vi "uRedPC.vi"() -> ()   [LabVIEW 2019]
uses:
  <vilib>/addons/_office/excel.llb/Excel Get Data ([dbl]).vi
  <vilib>/Utility/NIReport.llb/NI_report.lvclass
  <vilib>/Utility/NIReport.llb/Excel/NI_Excel.lvclass
  <vilib>/addons/_office/NI_ReportGenerationToolkit.lvlib
panel:
  out "Time":u32
  in  "Tab Control":enum32{"SoC", "Voltge-Current"}(tab)
  out "SoC Vehiculo":dbl[](graph)
  out "Battery Voltage":dbl[](graph)
  out "Battery Current":dbl[](graph)
  in  "%C":dbl=0.5 min=0.0 max=0.5 step=0.01
  out "Pot_cons":dbl
  out "V_bat":dbl
  out "I_bat":dbl
  in  "SoC0_Vehiculo":dbl=0.4 min=0.0 max=1.0 step=0.001
  in  "Cargar":bool
  in  "Boolean":bool
  out "Potencia consumida":dbl
  in  "Falla PV":bool
  in  "SoC_ini":dbl=0.5 min=0.0 max=1.0 step=0.1
  in  "Numero Paneles":u8=4 step=1
  in  "Voltaje Red":dbl=120.0 min=0.0 max=240.0 step=120.0
  out "Perdida Batería":dbl
  out "Perdida PV":dbl
  in  "Numero Baterías":u8=4 min=1 step=1
  out "Ring":u16(ring)
  out "Sheet 1 Data 2":dbl[][](array[numeric]) format="%.2f"
  out "Irradiancia":dbl(graph)
  out "Sheet 1 Data":dbl[][](array[numeric]) format="%.2f"
  out "SoC":dbl[](graph)
  out "Potencias":T1(graph)
  in  "stop":bool
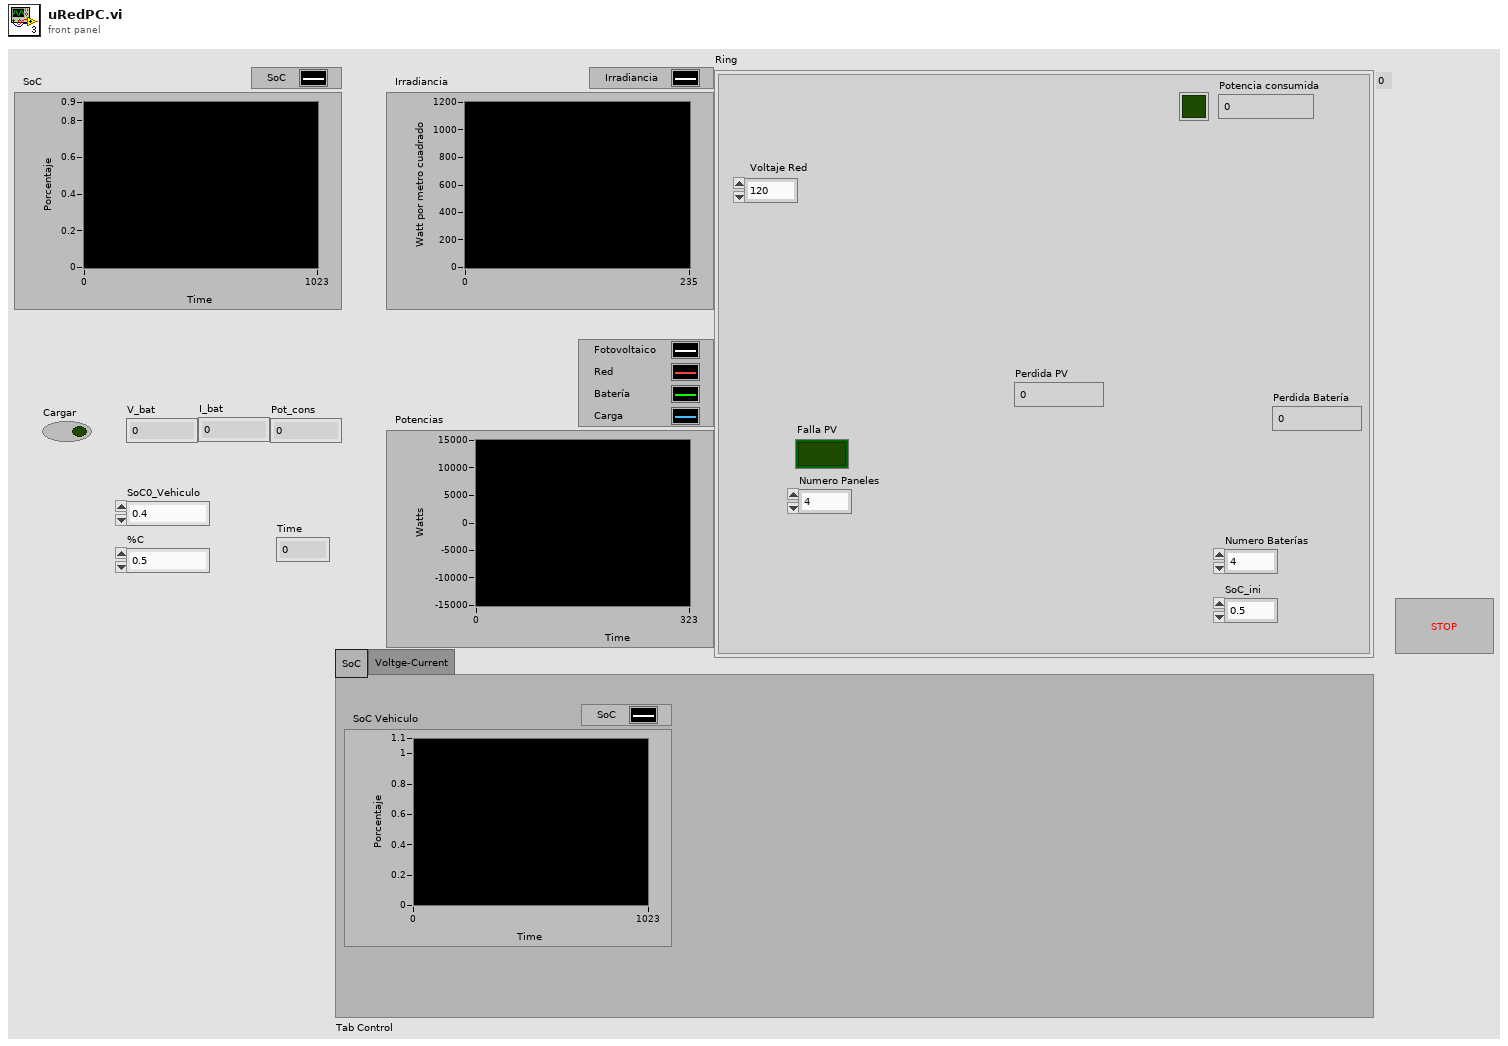
[diagram p1: front panel]
types:
  T1 = cluster{"Double":dbl, "Double":dbl, "Double":dbl, dbl}
  T2 = enum16{"Standard Report", "HTML", "Word", "Excel"}
  T3 = enum16{"open", "open or create", "create or replace", "create", "open (read-only)"}
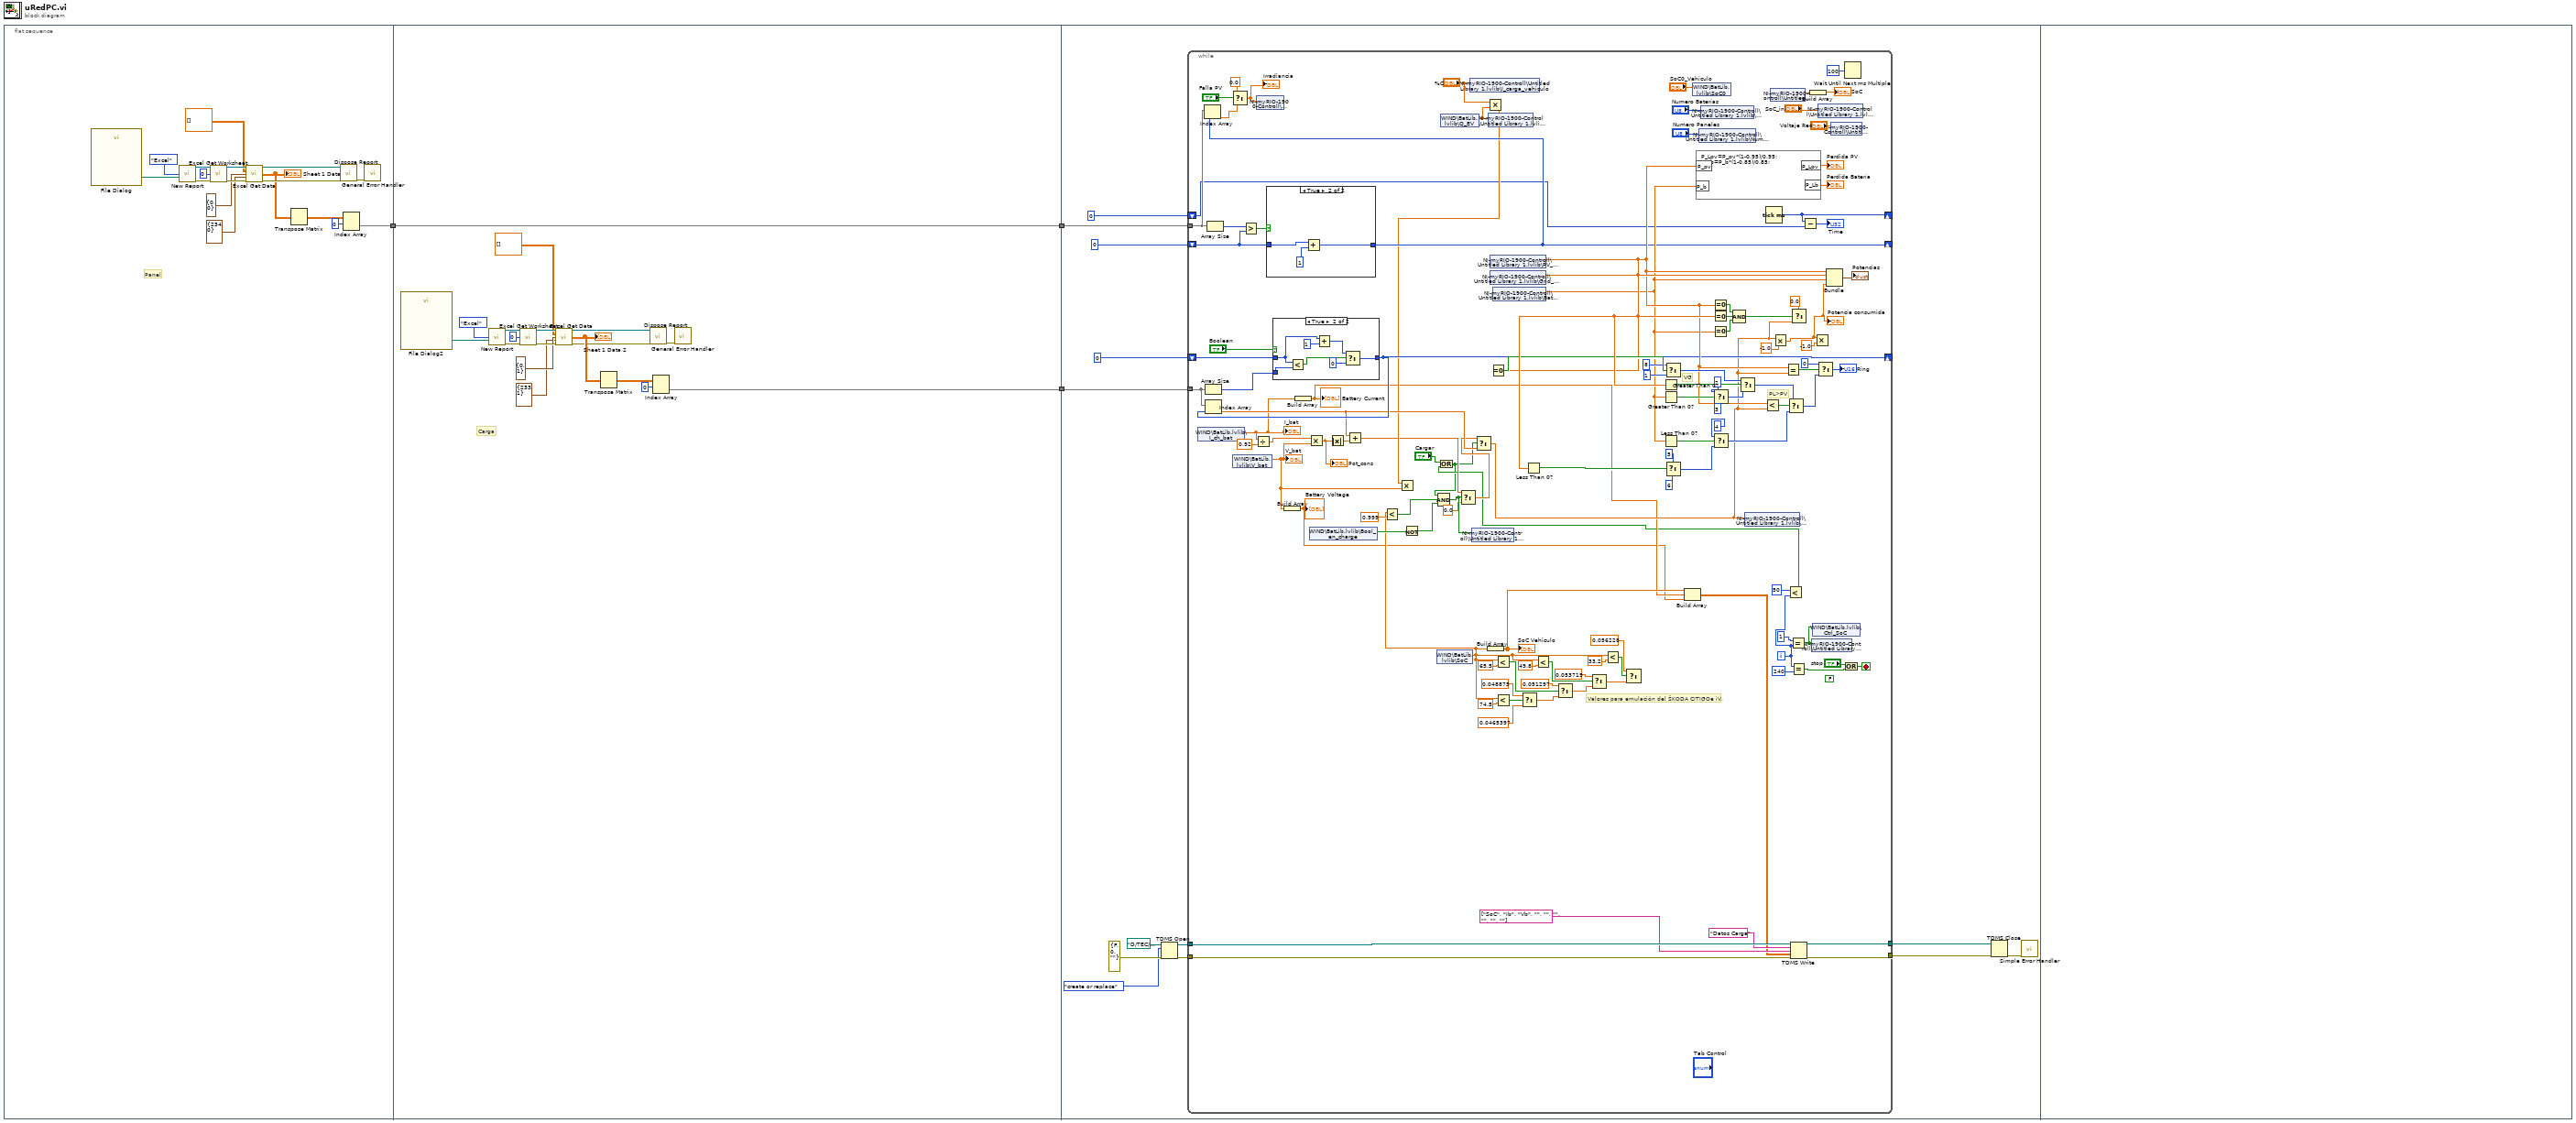
[diagram p0: block diagram]
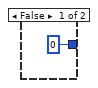
[diagram p3: hidden frame]
diagram:
  n1 = flat-sequence {
    tunnel: [w4] -> w3
    tunnel: [w38] -> w2
    tunnel: [w37] -> w1
    tunnel: w3 -> [w38]
    tunnel: w2 -> [w51]
    tunnel: w1 -> [w49]
    frame #0 {
      # "Panel"
      n2 = call "File Dialog"() -> ("selected path"=w11:path)  [unwired: 7 in, 8 out]
      n3 = call <vilib>:"New Report.vi"("report type"=T2."Excel", "template (empty)"=w11) -> ("report out"=w20:refnum<class "NI_report.lvclass">, "error out"=w16:errorcluster)  [unwired: 4 in, 8 out]
      n4 = call <vilib>:"Excel Get Worksheet.vi"("report in"=w20, "worksheet index (0)"=0, "error in (no error)"=w16) -> ("report out"=w19:refnum<class "NI_report.lvclass">, "error out"=w15:errorcluster)  [unwired: 11 out]
      n5 = call-poly <vilib>:"Excel Get Data.vi"("report in"=w19, "data type"=dbl[][] [], "start (-1, -1)"=cluster{"row":i32, "column":i32} {"row"=0, "column"=0}, "end (-1, -1)"=cluster{"row":i32, "column":i32} {"row"=234, "column"=0}, "error in (no error)"=w15) -> ("report out"=w10:refnum<class "NI_report.lvclass">, "data"=w7:dbl[][], "error out"=w9:errorcluster)  [unwired: 8 out]
      "Sheet 1 Data" <- w7
      n6 = Transpose Matrix(1:w7) -> (0:w6:dbl[][])
      n7 = call-dynamic "Dispose Report.vi"("report in"=w10, "error in (no error)"=w9) -> ("error out"=w12:errorcluster)  [unwired: 3 in, 10 out]
      n8 = Index Array(array=w6, index (row)=0) -> (element=w4:dbl[])  [unwired: 1 in]
      n9 = call <vilib>:"General Error Handler.vi"("error in (no error)"=w12) -> ()  [unwired: 3 in, 12 out]
    }
    frame #1 {
      # "Carga"
      n10 = call "File Dialog2"() -> ("selected path"=w32:path)  [unwired: 7 in, 8 out]
      n11 = call <vilib>:"New Report.vi"("report type"=T2."Excel", "template (empty)"=w32) -> ("report out"=w27:refnum<class "NI_report.lvclass">, "error out"=w29:errorcluster)  [unwired: 4 in, 8 out]
      n12 = call <vilib>:"Excel Get Worksheet.vi"("report in"=w27, "worksheet index (0)"=0, "error in (no error)"=w29) -> ("report out"=w28:refnum<class "NI_report.lvclass">, "error out"=w30:errorcluster)  [unwired: 11 out]
      n13 = call-poly <vilib>:"Excel Get Data.vi"("report in"=w28, "data type"=dbl[][] [], "start (-1, -1)"=cluster{"row":i32, "column":i32} {"row"=0, "column"=1}, "end (-1, -1)"=cluster{"row":i32, "column":i32} {"row"=233, "column"=1}, "error in (no error)"=w30) -> ("report out"=w33:refnum<class "NI_report.lvclass">, "data"=w35:dbl[][], "error out"=w34:errorcluster)  [unwired: 8 out]
      "Sheet 1 Data 2" <- w35
      n14 = Transpose Matrix(1:w35) -> (0:w36:dbl[][])
      n15 = call-dynamic "Dispose Report.vi"("report in"=w33, "error in (no error)"=w34) -> ("error out"=w31:errorcluster)  [unwired: 3 in, 10 out]
      n16 = Index Array(array=w36, index (row)=0) -> (element=w37:dbl[])  [unwired: 1 in]
      n17 = call <vilib>:"General Error Handler.vi"("error in (no error)"=w31) -> ()  [unwired: 3 in, 12 out]
    }
    frame #2 {
      n18 = TDMS Open(8:errorcluster {"status"=FALSE, "code"=0, "source"=""} ("error in (no error)"), 10:T3."create or replace" ("operation (0:open)"), 11:path "D:/TEC/Doctorado/MyRIO/uR_AC_V2/Datos_sims/Prueba.tdms" ("file path")) -> (0:w41:errorcluster, 3:w42:refnum<k34>)  [unwired: 4 in]
      n19 = while {
        tunnel: w51 -> [w164]
        shift-right: [w122] -> _
        shift-left: 0 -> [w161]
        tunnel: w49 -> [w165]
        shift-right: [w123] -> _
        shift-left: 0 -> [w162]
        shift-right: [w78] -> _
        shift-left: u32 0 ("millisecond timer value") -> [w77]
        tunnel: w42 -> [w71]
        tunnel: w41 -> [w70]
        tunnel: [w69] -> w40
        tunnel: [w68] -> w39
        i -> [w52]
        stop <- w114 stop-if-true
        (unwired) FALSE ("y")
        # "Valores para emulación del ŠKODA CITIGOe iV."
        # "VG"
        # "PL>PV"
        n20 = shared-variable "WIND\\BatLib.lvlib\\I_ch_bat"() -> (w74:dbl)  [unwired: 1 in, 1 out]
        "I_bat" <- w74
        n21 = Array Size(array=w165) -> (size(s)=w124:i32)
        n22 = Array Size(array=w164) -> (size(s)=w121:i32)
        n23 = shared-variable "WIND\\BatLib.lvlib\\V_bat"() -> (w73:dbl)  [unwired: 1 in, 1 out]
        "V_bat" <- w73
        n24 = Greater?(x=w121, y=w161) -> (0:w120:bool)
        n25 = Divide(x=w74, y=0.92) -> (x/y=w88:dbl)
        n26 = case shown="True" w120 {
          tunnel: [0 w179] -> w122
          tunnel: w161 -> [_ w180]
          frame False {
          }
          frame True {
            n27 = Add(x=w180, y=1) -> (x+y=w179:i32)
          }
        }
        n28 = Index Array(array=w164, index=w122) -> (element=w163:dbl)
        n29 = Select(t=0.0, s="Falla PV", f=w163) -> (s? t:f=w159:dbl)
        "Irradiancia" <- w159
        n30 = shared-variable "NI-myRIO-1900-Controll\\Untitled Library 1.lvlib\\G"(w159) -> ()  [unwired: 1 in, 1 out]
        n31 = case shown="True" "Boolean" {
          tunnel: [w170 w173] -> w123
          tunnel: w124 -> [_ w172]
          tunnel: w162 -> [w170 w171]
          frame False {
          }
          frame True {
            n32 = Less?(x=w171, y=w172) -> (x < y?=w176:bool)
            n33 = Add(x=w171, y=1) -> (x+y=w174:i32)
            n34 = Select(t=w174, s=w176, f=0) -> (s? t:f=w173:i32)
          }
        }
        n35 = Index Array(array=w165, index=w123) -> (element=w110:dbl)
        n36 = Build Array(w73) -> (w63:dbl[])
        "Battery Voltage" <- w63
        n37 = Build Array(w74) -> (w64:dbl[])
        "Battery Current" <- w64
        n38 = Multiply(x=w88, y=w73) -> (x*y=w109:dbl)
        "Pot_cons" <- w109
        n39 = shared-variable "WIND\\BatLib.lvlib\\Bool_en_charge"() -> (w83:bool)  [unwired: 1 in, 1 out]
        n40 = Absolute Value(x=w109) -> (abs(x)=w108:dbl)
        n41 = Add(x=w110, y=w108) -> (x+y=w59:dbl)
        n42 = Not(x=w83) -> (.not. x?=w82:bool)
        n43 = shared-variable "WIND\\BatLib.lvlib\\SoC"() -> (w72:dbl)  [unwired: 1 in, 1 out]
        n44 = Less?(x=w72, y=0.999) -> (x < y?=w61:bool)
        n45 = shared-variable "WIND\\BatLib.lvlib\\Q_EV"() -> (w86:dbl)  [unwired: 1 in, 1 out]
        n46 = shared-variable "NI-myRIO-1900-Controll\\Untitled Library 1.lvlib\\I_carga_vehiculo"("%C") -> ()  [unwired: 1 in, 1 out]
        n47 = Multiply(x="%C", y=w86) -> (x*y=w84:dbl)
        n48 = Multiply(x=w84, y=w73) -> ()  [unwired: 1 out]
        n49 = Build Array(w72) -> (w65:dbl[])
        "SoC Vehiculo" <- w65
        n50 = shared-variable "NI-myRIO-1900-Controll\\Untitled Library 1.lvlib\\Qch_EV"(w86) -> ()  [unwired: 1 in, 1 out]
        n51 = shared-variable "NI-myRIO-1900-Controll\\Untitled Library 1.lvlib\\Grid_Power"() -> (w140:dbl)  [unwired: 1 in, 1 out]
        n52 = shared-variable "NI-myRIO-1900-Controll\\Untitled Library 1.lvlib\\PV_POWER"() -> (w128:dbl)  [unwired: 1 in, 1 out]
        n53 = Equal To 0?(x=w128) -> (x = 0?=w132:bool)
        n54 = shared-variable "NI-myRIO-1900-Controll\\Untitled Library 1.lvlib\\Bat_Power"() -> (w127:dbl)  [unwired: 1 in, 1 out]
        n55 = Less?(x=w72, y=65.5) -> (x < y?=w103:bool)
        n56 = Less?(x=w72, y=74.5) -> (x < y?=w102:bool)
        n57 = Select(t=0.048875, s=w102, f=0.0465397) -> (s? t:f=w92:dbl)
        n58 = Less Than 0?(x=w140) -> (x < 0?=w139:bool)
        n59 = Less?(x=w72, y=49.8) -> (x < y?=w104:bool)
        n60 = Select(t=0.051297, s=w103, f=w92) -> (s? t:f=w94:dbl)
        n61 = Select(t=0.053719, s=w104, f=w94) -> (s? t:f=w96:dbl)
        n62 = Less?(x=w72, y=33.2) -> (x < y?=w105:bool)
        n63 = Select(t=0.056228, s=w105, f=w96) -> ()  [unwired: 1 out]
        n64 = Greater Than 0?(x=w140) -> (x > 0?=w148:bool)
        n65 = Greater Than 0?(x=w127) -> (x > 0?=w147:bool)
        n66 = Less Than 0?(x=w127) -> (x < 0?=w142:bool)
        n67 = Select(t=u16 8, s=w132, f=u16 1 ("t")) -> (s? t:f=w129:u16)
        n68 = Select(t=u16 5, s=w139, f=u16 6) -> (s? t:f=w134:u16)
        n69 = Build Array(w65, w64, w63) -> (w62:dbl[][])
        n70 = shared-variable "WIND\\BatLib.lvlib\\SoC0"("SoC0_Vehiculo") -> ()  [unwired: 1 in, 1 out]
        n71 = formula code="P_Lpv=P_pv*(1-0.95)/0.95;\nP_Lb=P_b*(1-0.85)/0.85;"("P_pv"=w128, "P_b"=w127) -> ("P_Lpv"=→"Perdida PV":dbl, "P_Lb"=→"Perdida Batería":dbl)
        n72 = shared-variable "NI-myRIO-1900-Controll\\Untitled Library 1.lvlib\\Num_Panel"("Numero Paneles") -> ()  [unwired: 1 in, 1 out]
        n73 = shared-variable "NI-myRIO-1900-Controll\\Untitled Library 1.lvlib\\Num_Bats"("Numero Baterías") -> ()  [unwired: 1 in, 1 out]
        n74 = Equal To 0?(x=w128) -> (x = 0?=w156:bool)
        n75 = Equal To 0?(x=w140) -> (x = 0?=w155:bool)
        n76 = Equal To 0?(x=w127) -> (x = 0?=w154:bool)
        n77 = Select(t=u16 2, s=w147, f=u16 3) -> (s? t:f=w144:u16)
        n78 = Select(t=u16 4, s=w142, f=w134) -> (s? t:f=w133:u16)
        n79 = Compound Arithmetic op=AND(w156, w155, w154) -> (w153:bool)
        n80 = Select(t=w129, s=w148, f=w144) -> (s? t:f=w143:u16)
        n81 = Tick Count (ms)() -> (millisecond timer value=w78:u32)
        n82 = shared-variable "NI-myRIO-1900-Controll\\Untitled Library 1.lvlib\\SoC"() -> (w168:dbl)  [unwired: 1 in, 1 out]
        n83 = Less?(x=50, y=w52) -> (x < y?=w54:bool)
        n84 = Or(x="Cargar", y=w54) -> (x .or. y?=w53:bool)
        n85 = Compound Arithmetic op=AND(w53, w61, w82) -> (w60:bool)
        n86 = Select(t=w59, s=w60, f=0.0) -> (s? t:f=w80:dbl)
        n87 = shared-variable "NI-myRIO-1900-Controll\\Untitled Library 1.lvlib\\Cargar"(w60) -> ()  [unwired: 1 in, 1 out]
        n88 = Select(t=w80, s=w53, f=w110) -> (s? t:f=w79:dbl)
        n89 = shared-variable "NI-myRIO-1900-Controll\\Untitled Library 1.lvlib\\LoadPower"(w79) -> ()  [unwired: 1 in, 1 out]
        n90 = Less?(x=w128, y=w79) -> (x < y?=w149:bool)
        n91 = Multiply(x=w79, y=-1.0) -> (x*y=w87:dbl)
        "Potencia consumida" <- w87
        n92 = Equal?(x=w128, y=w79) -> (x = y?=w151:bool)
        n93 = Select(t=w143, s=w149, f=w133) -> (s? t:f=w136:u16)
        n94 = Equal?(x=1, y=w52) -> (x = y?=w113:bool)
        n95 = Equal?(x=w52, y=240 ("x")) -> (x = y?=w75:bool)
        n96 = TDMS Write(0:w71, 5:"Datos Carga" ("group name in (Untitled)"), 7:string[] ["SoC", "Ib", "Vb", "", "", "", "", "", ""] ("channel name(s) in (Untitled)"), 9:w62, 11:w70) -> (4:w69:refnum<k34>, 15:w68:errorcluster)  [unwired: 1 in, 2 out]
        n97 = Select(t=0.0, s=w153, f=w79) -> ()  [unwired: 1 out]
        n98 = Subtract(x=w78, y=w77) -> (x-y=→"Time":u32)
        n99 = Build Array(w168) -> (→"SoC":dbl[])
        n100 = shared-variable "NI-myRIO-1900-Controll\\Untitled Library 1.lvlib\\InSoC"(w113) -> ()  [unwired: 1 in, 1 out]
        n101 = shared-variable "WIND\\BatLib.lvlib\\Ctrl_SoC"(w113) -> ()  [unwired: 1 in, 1 out]
        n102 = Multiply(x=w87, y=-1.0) -> ()  [unwired: 1 out]
        n103 = Select(t=u16 0, s=w151, f=w136) -> (s? t:f=→"Ring":u16)
        n104 = shared-variable "NI-myRIO-1900-Controll\\Untitled Library 1.lvlib\\SoC_ini"("SoC_ini") -> ()  [unwired: 1 in, 1 out]
        n105 = Bundle("Double"=w128, "Double"=w140, "Double"=w127, w87) -> (→"Potencias":T1)  [unwired: 1 in]
        n106 = shared-variable "NI-myRIO-1900-Controll\\Untitled Library 1.lvlib\\VG"("Voltaje Red") -> ()  [unwired: 1 in, 1 out]
        n107 = Or(x="stop", y=w75) -> (x .or. y?=w114:bool)
        n108 = Wait Until Next ms Multiple(millisecond multiple=u32 100) -> ()  [unwired: 1 out]
      }
      n109 = TDMS Close(8:w39, 11:w40) -> (0:w43:errorcluster)  [unwired: 1 out]
      n110 = call <vilib>:"Simple Error Handler.vi"("error in (no error)"=w43) -> ()  [unwired: 4 in, 5 out]
    }
    frame #3 {
    }
  }
